vi "Message distant perdu.vi"() -> ()   [LabVIEW 2022 SP3]
uses:
  Variables globales/Variable glob generale.vi
panel:
  out "Chemin":path
  in  "Bouton OK":bool
  # "la communication avec\nle poste distant :"
  # "a été perdue\nvérifier la liaison réseau"
  # "Ce logiciel et les informations qu'il contient, sont la propriété de l’IAS \net ne peuvent être diffusés sans l’autorisation de la Station d’étalonnage"
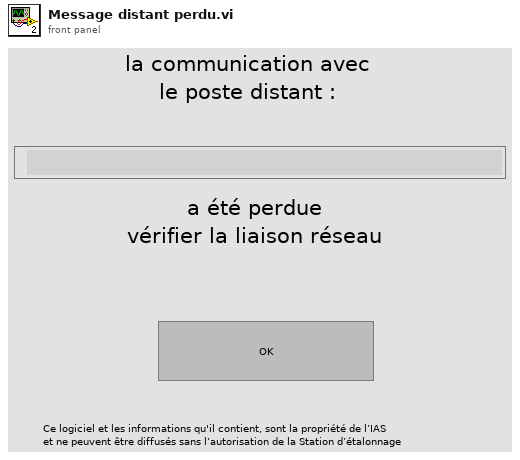
[diagram p1: front panel]
types:
  T1 = enum32{"Invalid", "Standard", "Closed", "Hidden", "Minimized", "Maximized"}
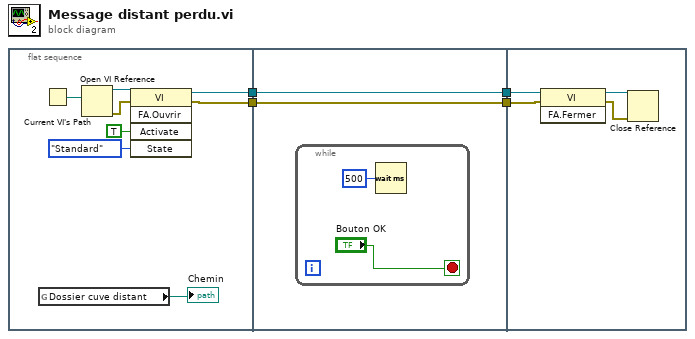
[diagram p0: block diagram]
diagram:
  n1 = flat-sequence {
    tunnel: [w9] -> w4
    tunnel: [w7] -> w1
    tunnel: w4 -> [w14]
    tunnel: [w14] -> w3
    tunnel: [w13] -> w2
    tunnel: w1 -> [w13]
    tunnel: w3 -> [w20]
    tunnel: w2 -> [w17]
    frame #0 {
      n2 = global read "Variable glob generale.vi" "Dossier cuve distant"() -> (→"Chemin":path)
      n3 = Current VI's Path() -> (path=w10:path)
      n4 = Open VI Reference(vi path=w10) -> (vi reference=w11:refnum<vi>, error out=w12:errorcluster)  [unwired: 5 in]
      n5 = invoke class="VI" method="FA.Ouvrir"(reference=w11, error in=w12, "Activate"=TRUE ("Activer ?"), "State"=T1."Standard" ("État")) -> (reference out=w9:refnum<vi>, error out=w7:errorcluster)  [unwired: 1 in, 3 out]
    }
    frame #1 {
      n6 = while {
        stop <- "Bouton OK" stop-if-true
        n7 = Wait (ms)(milliseconds to wait=u32 500 ("attente (ms)")) -> ()  [unwired: 1 out]
      }
    }
    frame #2 {
      n8 = invoke class="VI" method="FA.Fermer"(reference=w20, error in=w17) -> (reference out=w18:refnum<vi>, error out=w19:errorcluster)  [unwired: 1 in, 1 out]
      n9 = Close Reference(reference=w18, error in (no error)=w19) -> ()  [unwired: 1 out]
    }
  }
